vi "Validate Next State.vi"(7 "Normal State":T1, 8 "error in":errorcluster, 11 "Measure Call Context in":refnum<class "Measure Call Context.lvclass">) -> (0 "error out":errorcluster, 3 "measure call context out":refnum<class "Measure Call Context.lvclass">, 5 "Next State":T1)   [LabVIEW 2025, in "Automotive Ethernet Bus Monitor.lvclass"]
uses:
  Automotive Ethernet Bus Monitor.lvclass
  State.ctl
  <vilib>/Plug-In SDKs/Measurements/Measure Call Context/Measure Call Context.lvclass
  Automotive Ethernet Bus Monitor.lvclass/Automotive Ethernet Bus Monitor.ctl
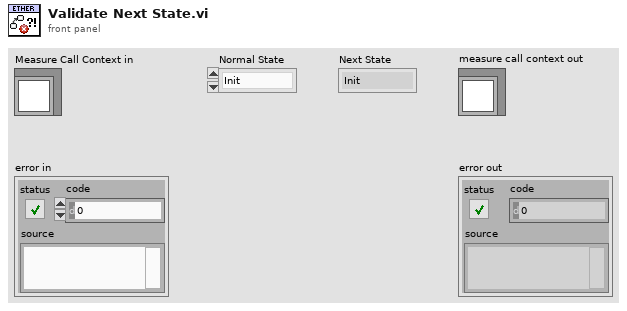
[diagram p1: front panel]
types:
  T1 = typedef "Automotive Ethernet Bus Monitor.lvclass/State.ctl" = enum16{"Init", "Execute", "Results", "Error", "Close"}
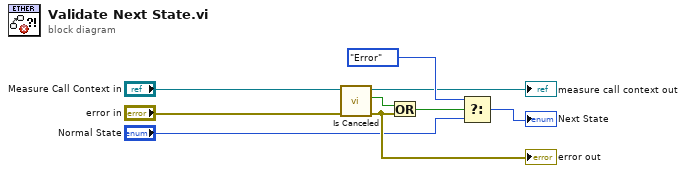
[diagram p0: block diagram]
diagram:
  n1 = call <vilib>:"Is Canceled.vi"("error in"="error in", "measure call context in"="Measure Call Context in") -> ("error out"=w9:errorcluster, "is canceled?"=w3:bool, "measure call context out"=→"measure call context out":refnum<class "Measure Call Context.lvclass">)  [unwired: 7 in]
  "error out" <- w9
  n2 = Or(x=w3, y=w9) -> (x .or. y?=w4:bool)
  n3 = Select(t=State."Error" ("State"), s=w4, f="Normal State") -> (s? t:f=→"Next State":T1)
